vi "Init.vi"(8 "error in (no error)":errorcluster, 10 "Instrument String":variant, 11 "NI DIO in":refnum<class "NI DIO.lvclass">) -> (0 "error out":errorcluster, 2 "Found?":bool=TRUE, 3 "NI DIO out":refnum<class "NI DIO.lvclass">)   [LabVIEW 2025, in "Digital IO.lvlib" / "NI DIO.lvclass"]
uses:
  NI DIO.lvclass
  NI DIO.lvclass/NI DIO.ctl
  Digital IO Channel/Digital IO Channel.lvclass
  Digital IO Channel configuration/Digital IO Channel configuration.lvclass
  Users/Public/Documents/Sandia National Labs/TSS Plugin/Abstract Engine.lvlibp/Abstract Instrument/Channel.ctl
  Users/Public/Documents/Sandia National Labs/TSS Plugin/Abstract Engine.lvlibp/Abstract Instrument/Data Type.ctl
  Digital IO Channel configuration/Digital IO Channel configuration.lvclass/Digital IO Channel configuration.ctl
  Digital IO Channel configuration/Read DIO Channel Setting.vi
  Users/Public/Documents/Sandia National Labs/TSS Plugin/CEF.lvlibp/Node/ReadChildren.vi
  Users/Public/Documents/Sandia National Labs/TSS Plugin/Abstract Engine.lvlibp/Channel configuration/Read Channel Setting.vi
  Users/Public/Documents/Sandia National Labs/TSS Plugin/CEF.lvlibp/Node/CEF_Node.lvclass
  Users/Public/Documents/Sandia National Labs/TSS Plugin/CEF.lvlibp/serializable configuration/CEF_serializable configuration.lvclass
  <vilib>/DAQmx/create/channels.llb/DAQmx Create Channel (DO-Digital Output).vi
  <vilib>/DAQmx/create/channels.llb/DAQmx Create Channel (DI-Digital Input).vi
  Users/Public/Documents/Sandia National Labs/TSS Plugin/Abstract Engine.lvlibp/Abstract Instrument/Abstract Instrument.lvclass
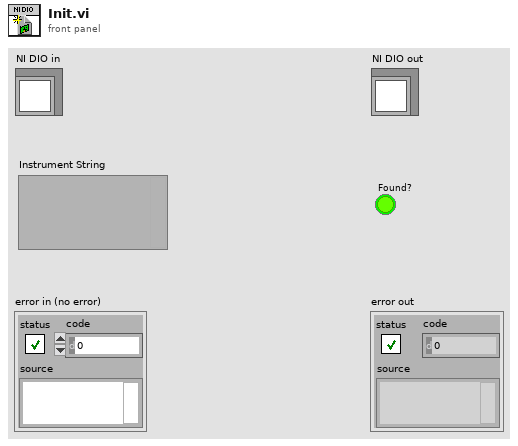
[diagram p1: front panel]
types:
  T1 = enum16{"---", "V", "A", "Ohm", "Hz", "uF", "degC", "deg"}
  T2 = typedef "Abstract Engine.lvlibp/Abstract Instrument.lvclass/Channel.ctl" = cluster{"Alias":string, "DataType":T3, "Unit":enum16{"---", "V", "A", "Ohm", "Hz", "uF", "degC", "deg"}, "Upper limit":dbl, "Lower limit":dbl, "Measurement":variant}
  T3 = typedef "Abstract Engine.lvlibp/Abstract Instrument.lvclass/Data Type.ctl" = string
  T4 = typedef "Abstract Engine.lvlibp/Channel configuration.lvclass/Default Channel.ctl" = cluster{"Address":string, "SW Alias":string, "Enabled":bool, "Type":string, "Description":string}
  T5 = typedef "Digital IO.lvlib/Digital IO Channel configuration.lvclass/DIO Channel Setting.ctl" = cluster{"Lines":string, "DataType":T3}
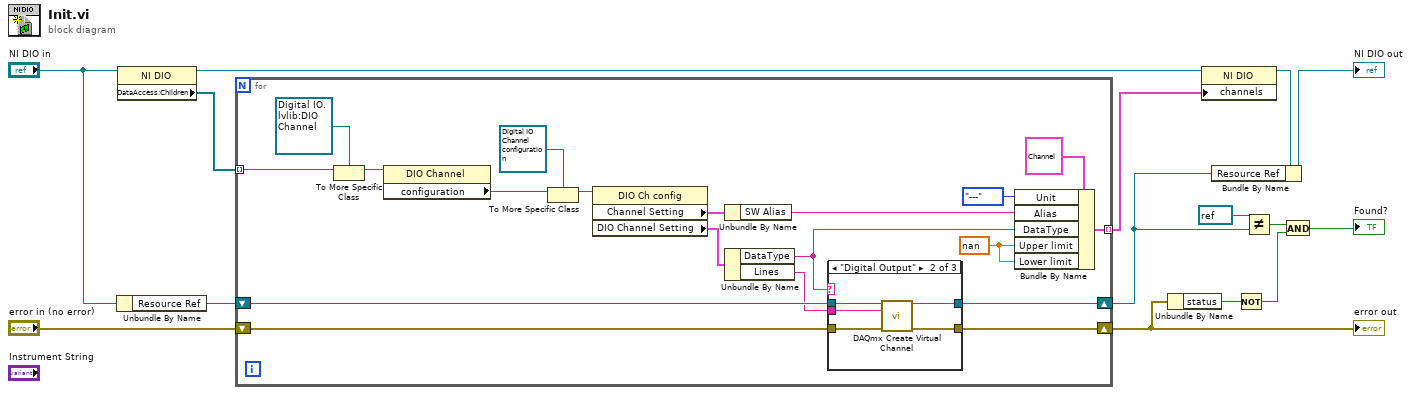
[diagram p0: block diagram]
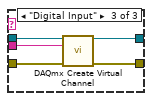
[diagram p3: hidden frame]
diagram:
  n1 = Unbundle By Name("NI DIO in") -> ("Resource Ref"=w5:refnum<k21>)
  n2 = property class="NI DIO"(reference="NI DIO in") -> (reference out=w14:refnum<class "NI DIO.lvclass">, "DataAccess:Children"=w4:refnum<data-value>[])  [unwired: 1 in, 1 out]
  n3 = for {
    shift-right: [w33] -> w10
    shift-left: w5 -> [w24]
    tunnel: w4 -> [w31] mode=indexing
    shift-right: [w34] -> w11
    shift-left: "error in (no error)" -> [w32]
    tunnel: [w20] -> w1 mode=indexing
    w21 = nan ("Upper limit")
    n4 = To More Specific Class(target class=refnum<data-value> refnum ("data value reference"), reference=w31) -> (specific class reference=w29:refnum<data-value>)  [unwired: 1 in, 1 out]
    n5 = property class="DIO Channel"(reference=w29) -> ("configuration"=w25:refnum<class "CEF_serializable configuration.lvclass">)  [unwired: 1 in, 2 out]
    n6 = To More Specific Class(target class=refnum<class "Digital IO Channel configuration.lvclass"> refnum ("Digital IO.lvlib:DIO Ch config"), reference=w25) -> (specific class reference=w27:refnum<class "Digital IO Channel configuration.lvclass">)  [unwired: 1 in, 1 out]
    n7 = property class="DIO Ch config"(reference=w27) -> ("Channel Setting"=w28:T4, "DIO Channel Setting"=w19:T5)  [unwired: 1 in, 2 out]
    n8 = Unbundle By Name(w28) -> ("SW Alias"=w18:string)
    n9 = Unbundle By Name(w19) -> ("DataType"=w17:T3, "Lines"=w16:string)
    n10 = case shown="\"Digital Output\"" w17 {
      tunnel: [w35 w41 w46] -> w34
      tunnel: [w36 w40 w45] -> w33
      tunnel: w32 -> [w35 w39 w44]
      tunnel: w24 -> [w36 w38 w43]
      tunnel: w16 -> [_ w37 w42]
      frame Default {
      }
      frame "Digital Output" {
        n11 = call-poly <vilib>:"DAQmx Create Virtual Channel.vi"("task in"=w38, "lines"=w37, "error in"=w39) -> ("task out"=w40:refnum<k21>, "error out"=w41:errorcluster)  [unwired: 11 in]
      }
      frame "Digital Input" {
        n12 = call-poly <vilib>:"DAQmx Create Virtual Channel.vi"("task in"=w43, "lines"=w42, "error in"=w44) -> ("task out"=w45:refnum<k21>, "error out"=w46:errorcluster)  [unwired: 11 in]
      }
    }
    n13 = Bundle By Name(cluster=T2 {"Alias"="ch0", "DataType"="Analog Input", "Unit"=enum."V", "Upper limit"=10.0, "Lower limit"=-10.0, "Measurement"=variant} ("Channel"), "Unit"=T1."---", "Alias"=w18, "DataType"=w17, "Upper limit"=w21, "Lower limit"=w21) -> (w20:T2)
  }
  "error out" <- w11
  n14 = Unbundle By Name(w11) -> ("status"=w13:bool)
  n15 = property class="NI DIO"(reference=w14, "channels"=w1) -> (reference out=w2:refnum<class "NI DIO.lvclass">)  [unwired: 1 in, 1 out]
  n16 = Bundle By Name(cluster=w2, "Resource Ref"=w10) -> (→"NI DIO out":refnum<class "NI DIO.lvclass">)
  n17 = Not(x=w13) -> (.not. x?=w12:bool)
  n18 = Not Equal?(x=refnum<k21> refnum, y=w10) -> (x != y?=w8:bool)
  n19 = And(x=w8, y=w12) -> (x .and. y?=→"Found?":bool)
